vi "Registration Mutex Name.vi"() -> (0 "registration semaphore name":string)   [LabVIEW 2018, in "GLog.lvlib" / "UI Updater.lvlib"]
uses:
  UI Updater.lvlib
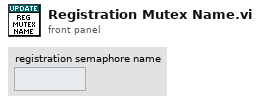
[diagram p1: front panel]
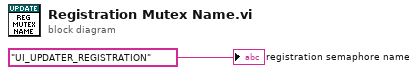
[diagram p0: block diagram]
diagram:
  "registration semaphore name" <- "UI_UPDATER_REGISTRATION" ("name (unnamed)")
